vi "Create_Data_For_WS2813.vi"(11 "Color Box":u32(colorbox)) -> (3 "string":string)   [LabVIEW 2025]
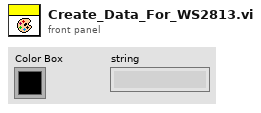
[diagram p1: front panel]
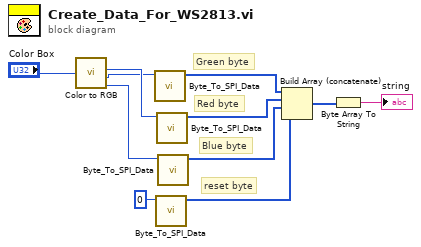
[diagram p0: block diagram]
diagram:
  # "reset byte"
  # "Blue byte"
  # "Red byte"
  # "Green byte"
  n1 = call <vilib>:"Color to RGB.vi"("Color"="Color Box") -> ("R"=w2:u8, "G"=w1:u8, "B"=w6:u8)  [unwired: 1 out]
  n2 = call "Byte_To_SPI_Data.vi"("Byte value"=w1) -> ("SPI Data"=w10:u8[])  [unwired: 10 in]
  n3 = call "Byte_To_SPI_Data.vi"("Byte value"=u8 0) -> ("SPI Data"=w3:u8[])  [unwired: 10 in]
  n4 = call "Byte_To_SPI_Data.vi"("Byte value"=w2) -> ("SPI Data"=w5:u8[])  [unwired: 10 in]
  n5 = call "Byte_To_SPI_Data.vi"("Byte value"=w6) -> ("SPI Data"=w4:u8[])  [unwired: 10 in]
  n6 = Build Array (concatenate)(w10, w5, w4, w3) -> (w11:u8[])
  n7 = Byte Array To String(unsigned byte array=w11) -> (string=→"string":string)
